vi "Delete.vi"(8 "error in":errorcluster, 10 "Path":path, 11 "IFile Manager in":refnum<class "Mock IFile Manager.lvclass">) -> (0 "error out":errorcluster, 3 "IFile Manager out":refnum<class "Mock IFile Manager.lvclass">)   [LabVIEW 2026, in "Mock IFile Manager.lvclass"]
doc: "Delete a file or folder without prompts."
uses:
  Mock IFile Manager.lvclass
  C:/Program Files/National Instruments/LabVIEW 2026/vi.lib/Astemes/LMock/Mock.lvclass
  Mock IFile Manager.lvclass/Mock IFile Manager.ctl
  <vilib>/Astemes/LMock/Mock.lvclass
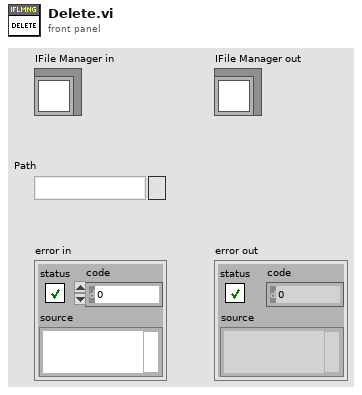
[diagram p1: front panel]
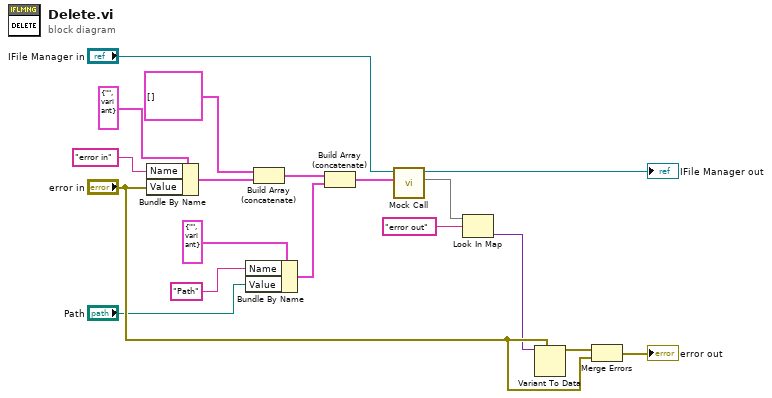
[diagram p0: block diagram]
diagram:
  n1 = Bundle By Name(cluster=cluster{"Name":string, "Value":variant} {"Name"="", "Value"=variant} ("element"), "Name"="error in", "Value"="error in") -> (w3:cluster{"Name":string, "Value":variant})
  n2 = Bundle By Name(cluster=cluster{"Name":string, "Value":variant} {"Name"="", "Value"=variant} ("element"), "Name"="Path", "Value"="Path") -> (w1:cluster{"Name":string, "Value":variant})
  n3 = Build Array (concatenate)(cluster{"Name":string, "Value":variant}[] [] ("Control Values"), w3) -> (w12:cluster{"Name":string, "Value":variant}[])
  n4 = Build Array (concatenate)(w12, w1) -> (w15:cluster{"Name":string, "Value":variant}[])
  n5 = call <vilib>:"Mock Call.vi"("Control Values"=w15, "Mock In"="IFile Manager in") -> ("Return Values"=w10:map{string, variant}, "Mock Out"=→"IFile Manager out":refnum<class "Mock IFile Manager.lvclass">)  [unwired: 8 in]
  n6 = Look In Map(map=w10, key="error out") -> (value=w8:variant)  [unwired: 1 in, 1 out]
  n7 = Variant To Data(type="error in", Variant=w8) -> (data=w7:errorcluster)  [unwired: 1 in, 1 out]
  n8 = Merge Errors(w7, "error in") -> (→"error out":errorcluster)
